vi "user32 ScreenToClient.vi"(0 "hWnd":u64, 5 "Screen X":i32, 7 "Screen Y":i32, 11 "error in (no error)":errorcluster) -> (4 "Client X":i32, 6 "Client Y":i32, 8 "return value":i32, 15 "error out":errorcluster)   [LabVIEW 2020, in "RemoteVI.lvlib"]
doc: "Converts a point from screen coordinates to the client coordinates of the window hWnd through user32.dll ScreenToClient (stdcall, called in any thread). The point travels to the DLL as a POINT {LONG x, LONG y} that the function overwrites in place. return value is the Win32 BOOL: non-zero on success, 0 on failure. When error in carries an error the DLL is not called. Generated by scripts\\Build Win32 Wrappers.vi - do not edit by hand, rebuild it."
uses:
  RemoteVI.lvlib
  user32.dll
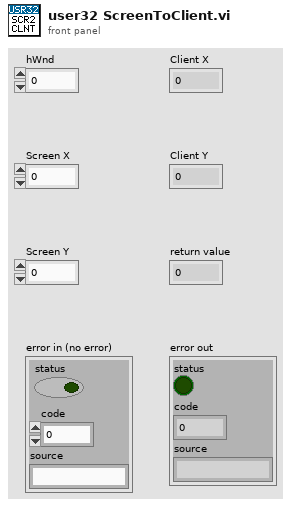
[diagram p1: front panel]
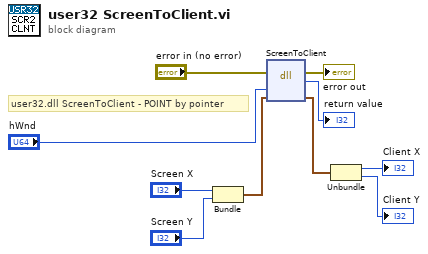
[diagram p0: block diagram]
diagram:
  # "user32.dll ScreenToClient - POINT by pointer"
  n1 = Bundle("Screen X"="Screen X", "Screen Y"="Screen Y") -> (w2:cluster{"Screen X":i32, "Screen Y":i32})  [unwired: 1 in]
  n2 = dll-call lib="user32.dll" fn="ScreenToClient"(error in="error in (no error)", "hWnd"="hWnd", "lpPoint"=w2) -> (error out=→"error out":errorcluster, →"return value":i32, "lpPoint"=w1:cluster{"Screen X":i32, "Screen Y":i32})  [unwired: 3 in, 1 out]
  n3 = Unbundle(w1) -> ("Screen X"=→"Client X":i32, "Screen Y"=→"Client Y":i32)
